vi "Turn.vi"(0 "T - 1st, F - 2nd":bool=TRUE, 1 "NXT/EV3 IN":T2, 2 "Motor IDs":cluster{"Motors":T1, "Motors 2":T1}={"Motors"=0, "Motors 2"=1} {"Motors 2" items=["Port A", "Port B", "Port C", "Port D"]; "Motors" items=["Port A", "Port B", "Port C", "Port D"]}, 3 "Power":dbl) -> (4 "NXT/EV3 OUT":T2)   [LabVIEW 2016, in "13.03 Robot.lvrbt"]
uses:
  13.03 Robot.lvrbt
  <vilib>/NXT/Subs/LVHSConnector.ctl
  <vilib>/NXT/LegoClasses/BrickReference/BrickReference.lvclass
  <vilib>/NXT/Block Support/NXT_OutputPort.ctl
  <vilib>/NXT/NXTIO Xnodes/NXTIONodeSubVIs/NXTMoveMotors.vi
  <vilib>/NXT/NXTIO Xnodes/NXTIOXNode/NXTIO.xnode
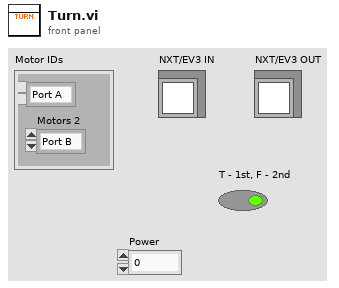
[diagram p1: front panel]
types:
  T1 = typedef "NXT_OutputPort.ctl" = u8
  T2 = typedef "LVHSConnector.ctl" = refnum<class "BrickReference.lvclass">
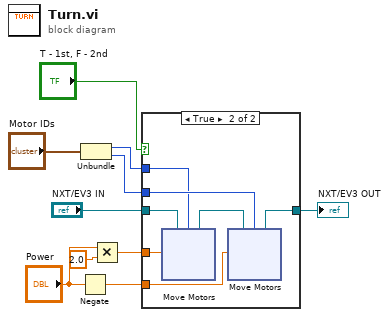
[diagram p0: block diagram]
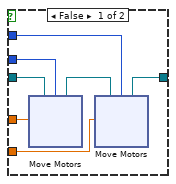
[diagram p2: hidden frame]
diagram:
  n1 = Negate(x="Power") -> (-x=w4:dbl)
  n2 = Unbundle("Motor IDs") -> ("Motors"=w2:T1, "Motors 2"=w3:T1)
  n3 = Multiply(x="Power", y=2.0) -> (x*y=w7:dbl)
  n4 = case shown="True" "T - 1st, F - 2nd" {
    tunnel: "NXT/EV3 IN" -> [w17 w38]
    tunnel: w7 -> [w14 w37]
    tunnel: w3 -> [w11 w36]
    tunnel: w4 -> [w15 w33]
    tunnel: [w13 w34] -> w6
    tunnel: w2 -> [w12 w32]
    frame False {
      n5 = xnode "Move Motors"("Power/Speed 1"=w14, "Motors"=w11, "NXT/EV3"=w17) -> ("NXT/EV3"=w16:T2)
      n6 = xnode "Move Motors"("Power/Speed 1"=w15, "Motors"=w12, "NXT/EV3"=w16) -> ("NXT/EV3"=w13:T2)
    }
    frame True {
      n7 = xnode "Move Motors"("Power/Speed 1"=w37, "Motors"=w32, "NXT/EV3"=w38) -> ("NXT/EV3"=w35:T2)
      n8 = xnode "Move Motors"("Power/Speed 1"=w33, "Motors"=w36, "NXT/EV3"=w35) -> ("NXT/EV3"=w34:T2)
    }
  }
  "NXT/EV3 OUT" <- w6
